vi "7. System-Level Module.vi"() -> ()   [LabVIEW 2017]
doc: "#### Overview\n\nDemonstrates how to create a system-level module and explains the difference between system-level modules and regular CSM modules when listing all active modules.\n\n#### Introduction\n\nSystem-level modules have a \".\" added as a prefix to their name, marking them as system-level modules. Functionally, system-level modules are identical to regular modules and can perform message communication and state registration. The difference is that system-level modules are not automatically listed in the active module list. This means that in normal logic scheduling, system-level modules will not be directly called and can only be triggered by explicit message transmission.\n\nTherefore, system-level modules are typically used to implement global background functions, such as scheduling modules in TCP programs.\n\nThis example demonstrates this distinction.\n\n#### Steps\n\n- Step1: Use the Advanced VIs to create a system-level module name by adding \".\" as a prefix to the CSM name. If you are familiar with the rules, you can also enter the corresponding name string and rule symbol directly without calling this API.\n- Step2: Synchronously call several \"regular\"/non-system-level CSM modules.\n- Step3: (Optional) Check if the CSM module name is valid. For more details, refer to the code of another example named `Module Naming Rules.vi`.\n- Step4: Wait for 1 second to ensure all modules finish starting.\n- Step5: List all active CSM modules. By default, system-level modules are not listed. By using the Advanced VIs, you can separate system-level modules from other regular modules for more efficient code development, debugging, etc.\n- Step6: Use unified logic to send the \"Macro:Exit\" message to all active regular CSM modules to stop them.\n- Step7: You can still send messages to system-level modules, such as sending the \"Macro:Exit\" message, to stop the system-level module."
uses:
  user.lib/_NEVSTOP/Communicable State Machine(CSM)/_Support/Error/CSM Invalid Name Error.vi
  user.lib/_NEVSTOP/Communicable State Machine(CSM)/Communicable State Machine.lvlib
panel:
  out "Module Names":string[](array[string])
  out "error out":errorcluster
  out "CSM Name(marked as Sysetem-Level Module)":string
  # "#CSM-Example Overview\n\nDemonstrates how to create a system-level module and explains the difference between system-level modules and regular CSM modules when listing all active modules."
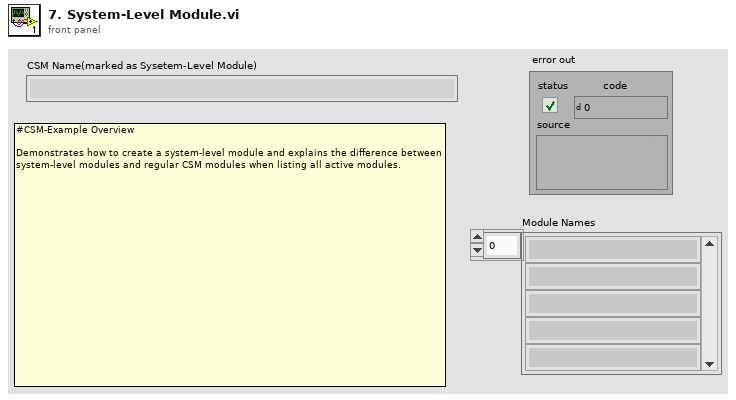
[diagram p1: front panel]
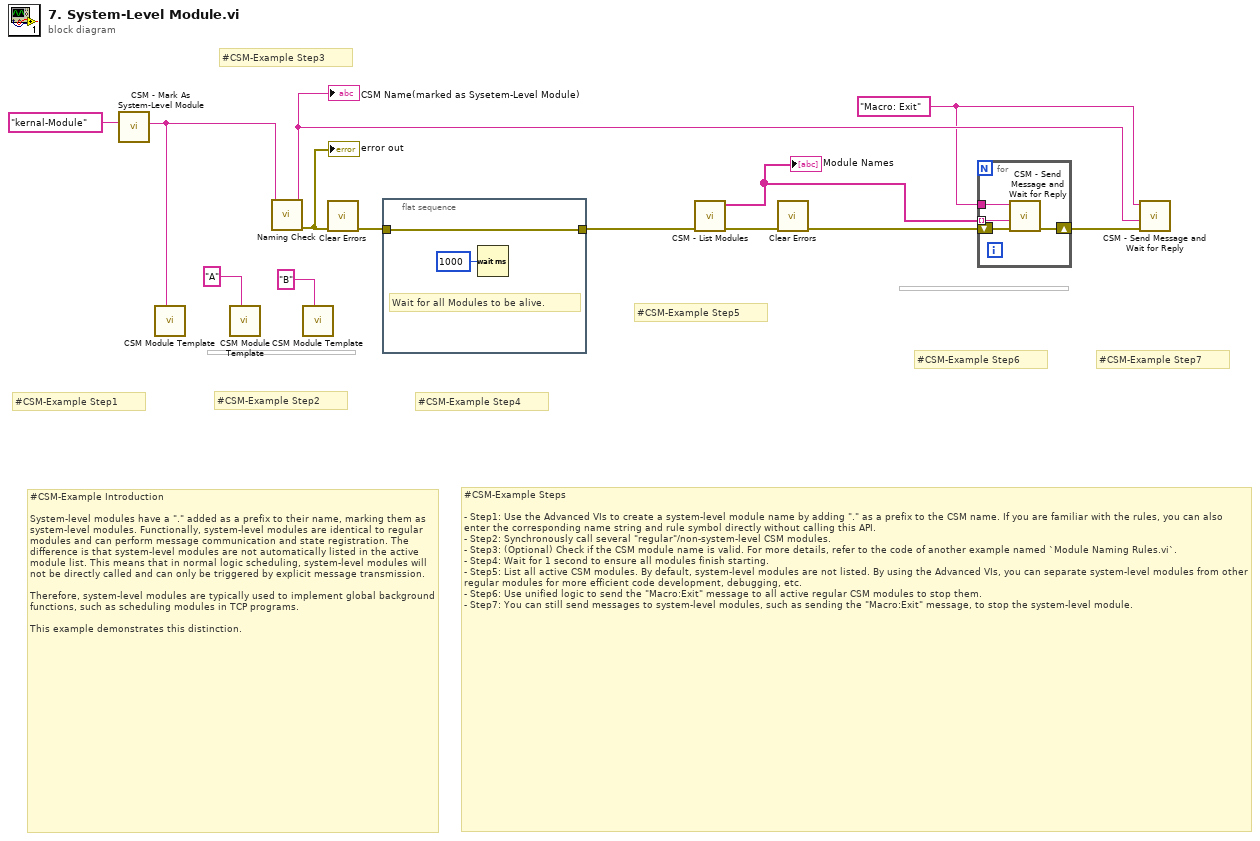
[diagram p0: block diagram]
diagram:
  w2 = "Macro: Exit" ("CSM Name")
  # "#CSM-Example Step7"
  # "#CSM-Example Step6"
  # "#CSM-Example Step5"
  # "#CSM-Example Step4"
  # "#CSM-Example Step3"
  # "#CSM-Example Step2"
  # "#CSM-Example Step1"
  # "#CSM-Example Steps\n\n- Step1: Use the Advanced VIs to create a system-level module name by adding \".\" as a prefix to the CSM name. If you are familiar with the rules, you can also enter the corresponding name string and rule symbol directly without calling this API.\n- Step2: Synchronously call several \"regular\"/non-system-level CSM modules.\n- Step3: (Optional) Check if the CSM module name is valid. For more details, refer to the code of another example named `Module Naming Rules.vi`.\n- Step4: Wait for 1 second to ensure all modules finish starting.\n- Step5: List all active CSM modules. By default, system-level modules are not listed. By using the Advanced VIs, you can separate system-level modules from other regular modules for more efficient code development, debugging, etc.\n- Step6: Use unified logic to send the \"Macro:Exit\" message to all active regular CSM modules to stop them.\n- Step7: You can still send messages to system-level modules, such as sending the \"Macro:Exit\" message, to stop the system-level module."
  # "#CSM-Example Introduction\n\nSystem-level modules have a \".\" added as a prefix to their name, marking them as system-level modules. Functionally, system-level modules are identical to regular modules and can perform message communication and state registration. The difference is that system-level modules are not automatically listed in the active module list. This means that in normal logic scheduling, system-level modules will not be directly called and can only be triggered by explicit message transmission.\n\nTherefore, system-level modules are typically used to implement global background functions, such as scheduling modules in TCP programs.\n\nThis example demonstrates this distinction."
  n1 = call "CSM - Mark As System-Level Module.vi"("CSM Name"="kernal-Module") -> ("CSM Name (Marked As Sysetem-Level Module)"=w12:string)  [unwired: 9 in]
  n2 = call "CSM Module Template.vi"("Name (\"\" to Use UUID)"=w12) -> ()  [unwired: 11 in]
  n3 = call "CSM Module Template.vi"("Name (\"\" to Use UUID)"="A" ("Name(\"\" to use uuid)")) -> ()  [unwired: 11 in]
  n4 = call "Naming Check.vi"("Name (\"\" to Use UUID)"=w12) -> ("error out"=w11:errorcluster, "Name (Dup)"=w7:string)  [unwired: 9 in]
  "CSM Name(marked as Sysetem-Level Module)" <- w7
  "error out" <- w11
  n5 = call "CSM Module Template.vi"("Name (\"\" to Use UUID)"="B" ("Name(\"\" to use uuid)")) -> ()  [unwired: 11 in]
  n6 = call <vilib>:"Clear Errors.vi"("error in (no error)"=w11) -> ("error out"=w9:errorcluster)  [unwired: 5 in, 1 out]
  n7 = flat-sequence {
    tunnel: [w14] -> w10
    tunnel: w9 -> [w14]
    frame #0 {
      # "Wait for all Modules to be alive."
      n8 = Wait (ms)(milliseconds to wait=u32 1000) -> ()  [unwired: 1 out]
    }
  }
  n9 = call "CSM - List Modules.vi"("Error In"=w10) -> ("error out"=w8:errorcluster, "Module Names"=w1:string[])  [unwired: 9 in]
  "Module Names" <- w1
  n10 = call <vilib>:"Clear Errors.vi"("error in (no error)"=w8) -> ("error out"=w6:errorcluster)  [unwired: 5 in, 1 out]
  n11 = for {
    tunnel: w2 -> [w17]
    shift-right: [w18] -> w5
    shift-left: w6 -> [w19]
    tunnel: w1 -> [w16] mode=indexing
    n12 = call "CSM - Send Message and Wait for Reply.vi"("Error In (No Error)"=w19, "Target Module"=w16, "State"=w17) -> ("error out"=w18:errorcluster)  [unwired: 6 in, 2 out]
  }
  n13 = call "CSM - Send Message and Wait for Reply.vi"("Error In (No Error)"=w5, "Target Module"=w7, "State"=w2) -> ()  [unwired: 6 in, 3 out]
